vi "PlaySubvi.vi"() -> ()   [LabVIEW 2025]
panel:
  in  "Enter your name":string
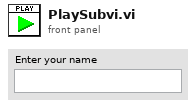
[diagram p1: front panel]
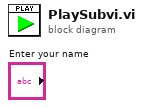
[diagram p0: block diagram]
diagram:
